vi "Test Batch Run with Broken Tests.vi"(8 "error in (no error)":errorcluster) -> (0 "error out":errorcluster)   [LabVIEW 2020]
uses:
  test-runner/test-brokenTests/Test Runner.BrokenTest.lvclass
  C:/projects/caraya/src/classes/Test Runner/Test Runner.lvclass
  classes/Test/Test.lvclass
  classes/Test Runner/Test Runner.lvclass
  classes/Assert/Assert.lvclass
panel:
  out "Test VIs":path[](array[path])
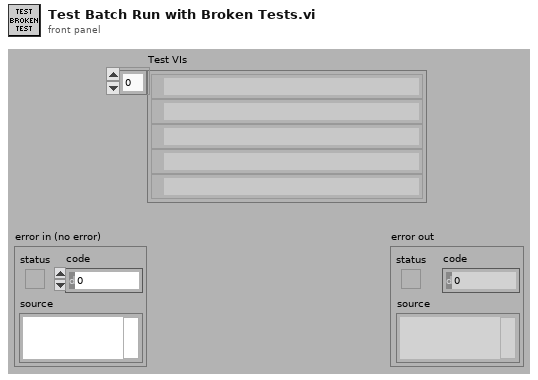
[diagram p1: front panel]
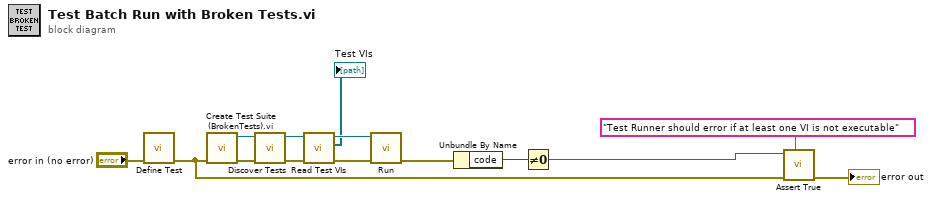
[diagram p0: block diagram]
diagram:
  n1 = call "Define Test.vi"("error in (no error)"="error in (no error)") -> ("error out"=w5:errorcluster)  [unwired: 9 in, 1 out]
  n2 = call "Create Test Suite (BrokenTests).vi.vi"("error in (no error)"=w5) -> ("error out"=w12:errorcluster, "Test Runner.BrokenTests"=w13:refnum<class "Test Runner.BrokenTest.lvclass">)  [unwired: 9 in]
  n3 = call "Discover Tests.vi"("error in (no error)"=w12, "Test Runner in"=w13) -> ("error out"=w9:errorcluster, "Test Runner out"=w11:refnum<class "Test Runner.BrokenTest.lvclass">)  [unwired: 8 in]
  n4 = call "Read Test VIs.vi"("error in (no error)"=w9, "Test Runner in"=w11) -> ("error out"=w8:errorcluster, "Test VIs"=→"Test VIs":path[], "Test Runner out"=w10:refnum<class "Test Runner.BrokenTest.lvclass">)  [unwired: 7 in]
  n5 = call "Run.vi"("error in (no error)"=w8, "Test Runner in"=w10) -> ("error out"=w2:errorcluster)  [unwired: 7 in, 2 out]
  n6 = Unbundle By Name(w2) -> ("code"=w6:i32)
  n7 = Not Equal To 0?(x=w6) -> (x != 0?=w4:bool)
  n8 = call "Assert True.vi"("Label"="Test Runner should error if at least one VI is not executable", "error in (no error)"=w5, "True?"=w4) -> ("error out"=→"error out":errorcluster)  [unwired: 7 in, 1 out]
